vi "Destroy Session.vi"(8 "error in (no error)":errorcluster, 11 "Session Handle":refnum<data-value>) -> (0 "error out":errorcluster)   [LabVIEW 2020, in "G-Embedded-Python-Interpreter-Toolkit.lvlib"]
uses:
  G-Embedded-Python-Interpreter-Toolkit.lvlib
  bin/gepit.cp310.32.dll
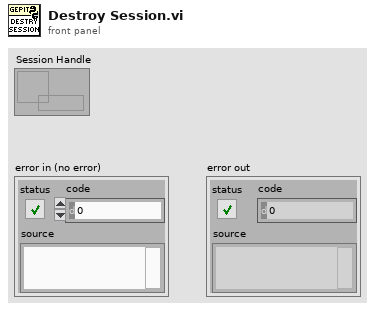
[diagram p1: front panel]
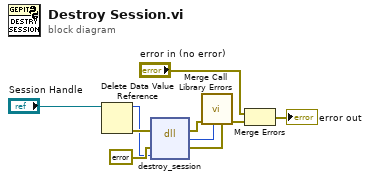
[diagram p0: block diagram]
diagram:
  n1 = Delete Data Value Reference(data value reference="Session Handle") -> (data value=w4:u64, error out=w5:errorcluster)  [unwired: 1 in]
  n2 = dll-call lib="C:/serenial/libraries/g-embedded-python-interpreter-toolkit/LabVIEW/bin/gepit.cp310.32.dll" fn="destroy_session"(error in=w5, "Error"=errorcluster {"status"=FALSE, "code"=0, "source"=""} ("error constant"), "Session"=w4) -> (error out=w9:errorcluster, "return type"=w8:i32, "Error"=w7:errorcluster)  [unwired: 3 in, 1 out]
  n3 = call "Merge Call Library Errors.vi"("Call Library Error"=w7, "Return Value"=w8, "error in"=w9) -> ("error out"=w3:errorcluster)  [unwired: 8 in]
  n4 = Merge Errors("error in (no error)", w3) -> (→"error out":errorcluster)
